vi "detect chassis.vi"() -> (0 "error out":errorcluster, 2 "passed?":bool)   [LabVIEW 2014, in "tests.lvlib"]
uses:
  tests.lvlib
  classes/SysCfg Device/SysCfg Device.lvclass
  classes/Controller/Controller.lvclass
  classes/Chassis/Chassis.lvclass
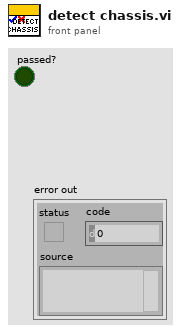
[diagram p1: front panel]
types:
  T1 = typedef "SMI.lvlib/Device.lvclass/login credentials.ctl" = cluster{"device class":string, "hostname":string, "IP address":string, "username":string, "password":string}
  T2 = typedef "SMI.lvlib/Chassis.lvclass/chassis and module information.ctl" = cluster{"chassis":T3, "modules":T4[]}
  T3 = typedef "SMI.lvlib/Chassis.lvclass/chassis information.ctl" = cluster{"resource name":string, "vendor name":string, "product name":string, "product ID":u16, "serial number":string, "number of slots":i32, "device class":string}
  T4 = typedef "SMI.lvlib/Module.lvclass/module information.ctl" = cluster{"vendor name":string, "product name":string, "product ID":u16, "serial number":string}
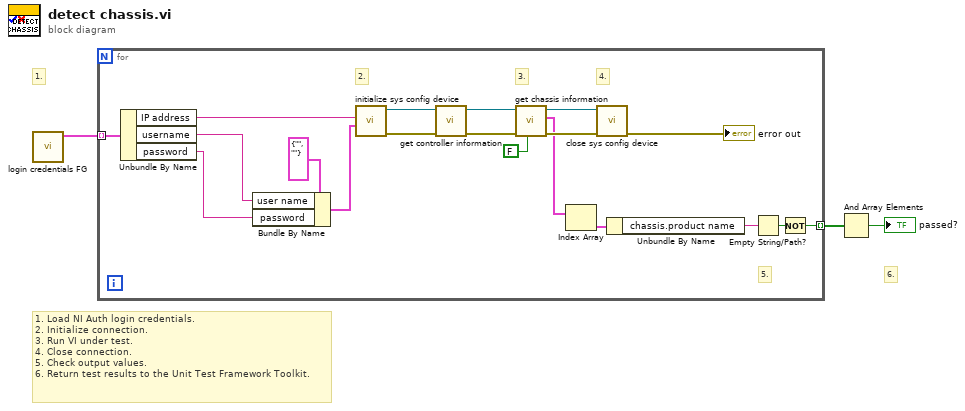
[diagram p0: block diagram]
diagram:
  # "1."
  # "6."
  # "1. Load NI Auth login credentials.\n2. Initialize connection.\n3. Run VI under test.\n4. Close connection.\n5. Check output values.\n6. Return test results to the Unit Test Framework Toolkit."
  n1 = call "login credentials FG.vi"() -> ("login credentials"=w1:T1[])  [unwired: 10 in, 1 out]
  n2 = for {
    tunnel: [w20] -> w2 mode=indexing
    tunnel: w1 -> [w8] mode=indexing
    # "4."
    # "2."
    # "3."
    # "5."
    n3 = Unbundle By Name(w8) -> ("IP address"=w7:string, "username"=w6:string, "password"=w5:string)
    n4 = Bundle By Name(cluster=cluster{"user name":string, "password":string} {"user name"="", "password"=""} ("login"), "user name"=w6, "password"=w5) -> (w9:cluster{"user name":string, "password":string})
    n5 = call "initialize sys config device.vi"("login"=w9, "IP address (localhost)"=w7) -> ("error out"=w22:errorcluster, "controller out"=w21:refnum<class "Controller.lvclass">)  [unwired: 8 in]
    n6 = call "get controller information.vi"("error in"=w22, "controller in"=w21) -> ("error out"=w17:errorcluster, "controller out"=w19:refnum<class "Controller.lvclass">)  [unwired: 7 in, 1 out]
    n7 = call "get chassis information.vi"("detect modules (T)"=FALSE, "error in"=w17, "controller in"=w19) -> ("error out"=w16:errorcluster, "local chassis"=w14:T2[], "controller out"=w18:refnum<class "Controller.lvclass">)  [unwired: 5 in, 1 out]
    n8 = Index Array(array=w14) -> (element=w13:T2)  [unwired: 1 in]
    n9 = call "close sys config device.vi"("error in"=w16, "controller in"=w18) -> ("error out"=→"error out":errorcluster)  [unwired: 8 in, 1 out]
    n10 = Unbundle By Name(w13) -> ("chassis.product name"=w12:string)
    n11 = Empty String/Path?(string/path=w12) -> (empty?=w11:bool)
    n12 = Not(x=w11) -> (.not. x?=w20:bool)
  }
  n13 = And Array Elements(Boolean array=w2) -> (logical AND=→"passed?":bool)
